vi "AssertSubpanelExecStateBad_Tests.vi"(11 "error in":errorcluster) -> (15 "error out":errorcluster)   [LabVIEW 2016, in "DronaTest.lvlib"]
uses:
  DronaTest.lvlib
  APIs/Stimulus/ControlValue/ValueSignalByPathString.vi
  APIs/Assert/AssertControlValue/Controls/Subpanel/AssertSubpanelVIExecBad.vi
  <vilib>/addons/_JKI Toolkits/Caraya/classes/Test/Test.lvclass
  Drona.lvlib
  APIs/Stimulus/ControlValue/ControlValue.lvlib
  APIs/Assert/AssertControlValue/Controls/Subpanel/AssertSubpanel.lvlib
  <vilib>/addons/_JKI Toolkits/Caraya/classes/Assert/Assert.lvclass
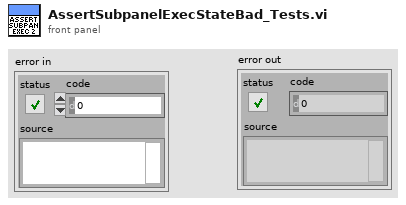
[diagram p1: front panel]
types:
  T1 = enum32{"Bad", "Idle", "Run top level", "Running"}
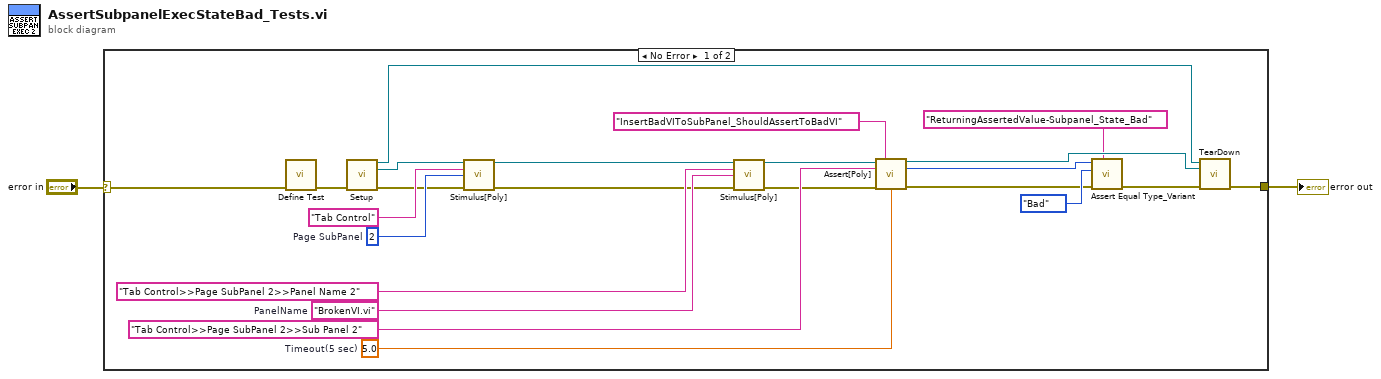
[diagram p0: block diagram]
diagram:
  n1 = case shown="No Error" "error in" {
    selector: "error in" -> [w24 w26]
    tunnel: [w11 w26] -> w1
    frame No Error {
      w15 = 2  # Page SubPanel
      w20 = "BrokenVI.vi"  # PanelName
      w21 = 5.0  # Timeout(5 sec)
      n2 = call <vilib>:"Define Test.vi"("error in (no error)"=w24) -> ("error out"=w17:errorcluster)  [unwired: 9 in, 1 out]
      n3 = call "Setup.vi"("error in"=w17) -> ("Application Ref"=w9:refnum<vi>, "VI out"=w8:refnum<vi>, "error out"=w12:errorcluster)  [unwired: 12 in]
      n4 = call-poly "Stimulus[Poly].vi"("VI Reference In"=w8, "Control Path"="Tab Control", "Value (Signaling)"=w15, "error in"=w12) -> ("VI Reference Out"=w18:refnum<vi>, "error out"=w14:errorcluster)  [unwired: 10 in]
      n5 = call-poly "Stimulus[Poly].vi"("VI Reference In"=w18, "Control Path"="Tab Control>>Page SubPanel 2>>Panel Name 2", "Value (Signaling)"=w20, "error in"=w14) -> ("VI Reference Out"=w13:refnum<vi>, "error out"=w19:errorcluster)  [unwired: 10 in]
      n6 = call-poly "Assert[Poly].vi"("VI Reference In"=w13, "Test Label"="InsertBadVIToSubPanel_ShouldAssertToBadVI" ("Label"), "Control Path"="Tab Control>>Page SubPanel 2>>Sub Panel 2", "Error In"=w19, "Timeout(5 sec)"=w21) -> ("VI Reference Out"=w10:refnum<vi>, "Asserted Value"=w3:T1, "Error Out"=w6:errorcluster)  [unwired: 8 in]
      n7 = call <vilib>:"Assert Equal Type_Variant.vi"("Label"="ReturningAssertedValue-Subpanel_State_Bad", "error in (no error)"=w6, "Y"=T1."Bad" ("Asserted Value"), "X"=w3) -> ("error out"=w5:errorcluster)  [unwired: 6 in, 1 out]
      n8 = call "TearDown.vi"("Application Ref"=w9, "VI in"=w10, "error in (no error)"=w5) -> ("error out"=w11:errorcluster)  [unwired: 12 in]
    }
    frame Error {
    }
  }
  "error out" <- w1
